vi "Prefilter.Low Pass.vi"(8 "error in (no error)":errorcluster, 9 "Low Pass Cutoff (Hz)":dbl, 10 "signal in":waveform(dbl)[](array[waveform]), 11 "DSP in":refnum<class "DSP.lvclass">) -> (0 "error out":errorcluster, 2 "signa out":waveform(dbl)[](array[waveform]), 3 "DSP out":refnum<class "DSP.lvclass">)   [LabVIEW 2019, in "DSP.lvclass"]
uses:
  DSP.lvclass
  DSP.lvclass/DSP.ctl
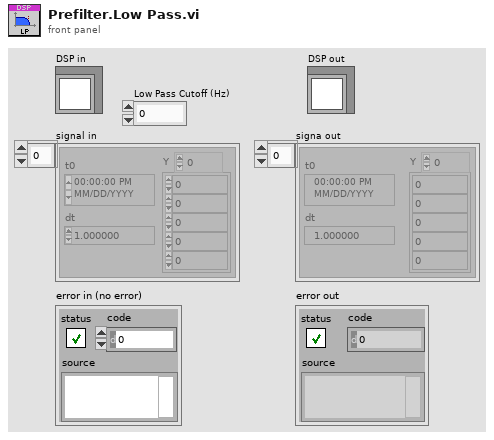
[diagram p1: front panel]
types:
  T1 = cluster{"filter structure":enum32{"IIR 2nd Order", "IIR 4th Order"}, "Reverse Coefficients":dbl[], "Forward Coefficients":dbl[]}[]
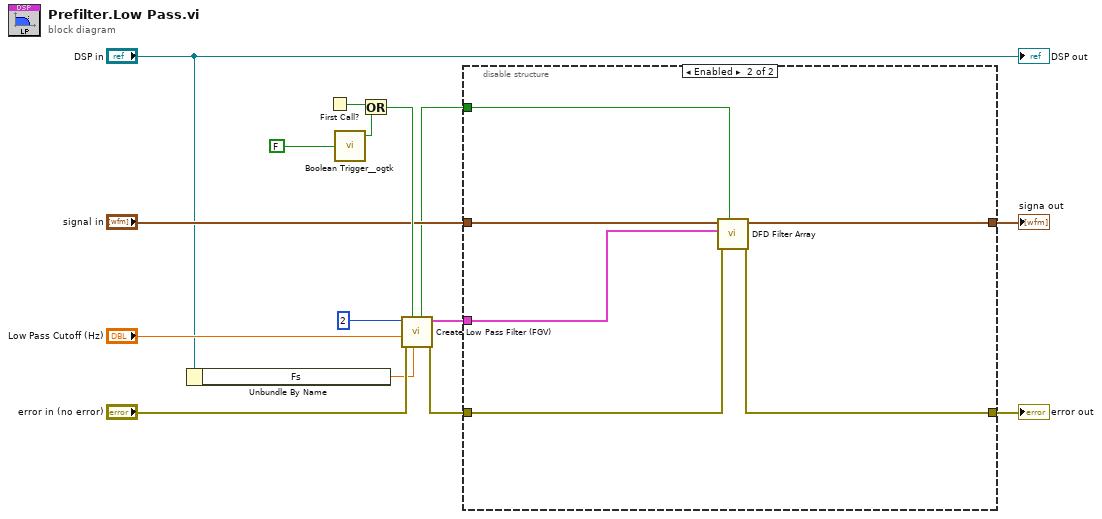
[diagram p0: block diagram]
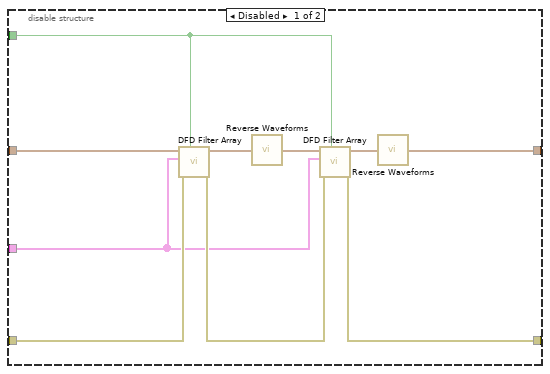
[diagram p2: hidden frame]
diagram:
  n1 = Unbundle By Name("DSP in") -> ("Fs"=w3:dbl)
  n2 = First Call?() -> (First Call?: T/F=w13:bool)
  n3 = call <userlib>:"Boolean Trigger__ogtk.vi"("Boolean Input"=FALSE) -> ("Rising Edge"=w12:bool)  [unwired: 1 in, 1 out]
  n4 = Or(x=w13, y=w12) -> (x .or. y?=w11:bool)
  n5 = call "Create Low Pass Filter (FGV).vi"("fs (Hz)"=w3, "init [F]"=w11, "error in (no error)"="error in (no error)", "Low Pass Cutoff (Hz)"="Low Pass Cutoff (Hz)", "order"=2) -> ("error out"=w7:errorcluster, "IIR Filters"=w1:T1, "init out"=w6:bool)  [unwired: 4 in]
  n6 = disable-structure shown="Enabled" {
    disable-tunnel: [w21 w27] -> w14
    disable-tunnel: w7 -> [w20 w28]
    disable-tunnel: w6 -> [w19 w30]
    disable-tunnel: [w18 w29] -> w9
    disable-tunnel: "signal in" -> [w17 w31]
    disable-tunnel: w1 -> [w16 w26]
    frame Disabled {
      n7 = call "DFD Filter Array.vi"("init (F)"=w19, "error in (no error)"=w20, "IIR Filters"=w16, "signal in"=w17) -> ("error out"=w22:errorcluster, "signal out"=w23:waveform(dbl)[])  [unwired: 6 in]
      n8 = call "Reverse Waveforms.vi"("signal in"=w23) -> ("Array"=w25:waveform(dbl)[])
      n9 = call "DFD Filter Array.vi"("init (F)"=w19, "error in (no error)"=w22, "IIR Filters"=w16, "signal in"=w25) -> ("error out"=w21:errorcluster, "signal out"=w24:waveform(dbl)[])  [unwired: 6 in]
      n10 = call "Reverse Waveforms.vi"("signal in"=w24) -> ("Array"=w18:waveform(dbl)[])
    }
    frame Enabled {
      n11 = call "DFD Filter Array.vi"("init (F)"=w30, "error in (no error)"=w28, "IIR Filters"=w26, "signal in"=w31) -> ("error out"=w27:errorcluster, "signal out"=w29:waveform(dbl)[])  [unwired: 6 in]
    }
  }
  "error out" <- w14
  "signa out" <- w9
  "DSP out" <- "DSP in"
